vi "Table Buffer - Destroy.vi"(8 "error in (no error)":errorcluster) -> (0 "error out":errorcluster)   [LabVIEW 2025, in "I2C Bus Monitor UI.lvlib"]
uses:
  I2C Bus Monitor UI.lvlib
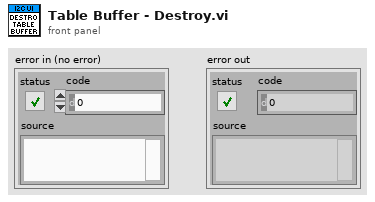
[diagram p1: front panel]
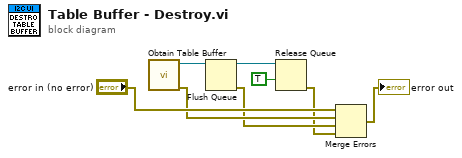
[diagram p0: block diagram]
diagram:
  n1 = call "Obtain Table Buffer.vi"() -> ("error out"=w3:errorcluster, "Table Queue"=w6:refnum<queue>)  [unwired: 10 in]
  n2 = Flush Queue(queue=w6) -> (queue out=w7:refnum<queue>, error out=w2:errorcluster)  [unwired: 1 in, 1 out]
  n3 = Release Queue(queue=w7, force destroy? (F)=TRUE) -> (error out=w1:errorcluster)  [unwired: 1 in, 2 out]
  n4 = Merge Errors("error in (no error)", w3, w2, w1) -> (→"error out":errorcluster)
